vi "RichToFlatcif_can_writer_cansub_GetCANStatusRequest.vi"(5 "OutputClusterType":T1, 11 "InputCluster":T2) -> (3 "OutputCluster":T1)   [LabVIEW 2021, in "CanWriterCansub_client.lvlib"]
uses:
  CanWriterCansub_client.lvlib
  cif_can_writer_cansub_GetCANStatusRequest.ctl
  cif_can_writer_cansub_GetCANStatusRequest_Flat.ctl
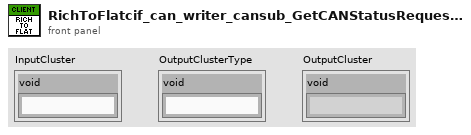
[diagram p1: front panel]
types:
  T1 = typedef "CanWriterCansub_client.lvlib/cif_can_writer_cansub_GetCANStatusRequest_Flat.ctl" = cluster{"void":string}
  T2 = typedef "CanWriterCansub_client.lvlib/cif_can_writer_cansub_GetCANStatusRequest.ctl" = cluster{"void":string}
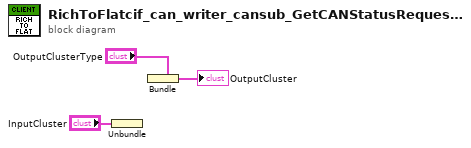
[diagram p0: block diagram]
diagram:
  n1 = Unbundle "Unbundle"("InputCluster") -> ()  [unwired: 1 out]
  n2 = Bundle "Bundle"(cluster="OutputClusterType") -> (→"OutputCluster":T1)  [unwired: 1 in]
